vi "Two Way Event Recorder RT Driver VI.vi"(6 "Device Clock":string, 9 "Device Inputs FIFO":refnum<k33>, 10 "Device Outputs FIFO":refnum<k33>, 11 "Device Reference":T1 format="%.0x") -> ()   [LabVIEW 2017, in "Two Way Event Recorder Custom Device.lvlib"]
uses:
  Two Way Event Recorder Custom Device.lvlib
  <vilib>/NI Veristand/Custom Device API/Custom Device Item Ref.ctl
  <vilib>/NI Veristand/Custom Device API/Custom Device Channel Type.ctl
  <vilib>/NI Veristand/Custom Device API/Custom Device Waveform DataType.ctl
  <vilib>/NI Veristand/Custom Device API/Message Response (String).ctl
  <vilib>/NI Veristand/Custom Device API/Message Response (Byte Array).ctl
  <vilib>/NI Veristand/Custom Device Waveform API/Waveform Session.lvclass/Waveform Session.ctl
  <vilib>/NI VeriStand/Custom Device Waveform API/Single Waveform Write (DBL)/Single Waveform Write (DBL).lvclass/Single Waveform Write (DBL).ctl
  <vilib>/NI Veristand/Custom Device Waveform API/Internal Comm Classes/WPL Comm/WPL Comm.lvclass/WPL Comm.ctl
  <vilib>/NI VeriStand/Custom Device Waveform API/Internal Comm Classes/WPL Comm/WPL Comm (1D DBL)/WPL Comm (1D DBL).lvclass/WPL Comm (1D DBL).ctl
  <vilib>/NI Veristand/Custom Device Waveform API/Single Waveform Write (DBL)/NI VeriStand - Start Single Waveform (DBL).vi
  <vilib>/NI Veristand/Custom Device Waveform API/Single Waveform Write (DBL)/NI VeriStand - Write Single Waveform (DBL).vi
  <vilib>/NI Veristand/Custom Device Waveform API/Internal Comm Classes/WPL Comm/WPL_start dbl waveform.vi
  <vilib>/NI Veristand/Custom Device Waveform API/Read Sample offset DVR.vi
  <vilib>/NI Veristand/Custom Device Waveform API/Check Opened.vi
  <vilib>/NI Veristand/Custom Device Waveform API/Internal Comm Classes/WPL Comm/WPL Comm (1D DBL)/Comm_write 1d dbl.vi
  <vilib>/NI Veristand/Custom Device Waveform API/Internal Comm Classes/WPL Comm/Set t0 on Variant.vi
  <vilib>/NI Veristand/Custom Device Waveform API/Internal Comm Classes/WPL Comm/Send WPL Command.vi
  <vilib>/NI Veristand/Custom Device Waveform API/Internal Comm Classes/WPL Comm/Direct Send WPL Command.vi
  <vilib>/NI Veristand/Custom Device Waveform API/Internal Comm Classes/WPL Comm/Convert Q Error to Shutdown Error.vi
  <vilib>/NI VeriStand/Custom Device Waveform API/Single Waveform Write (DBL)/Single Waveform Write (DBL).lvclass
  C:/Program Files (x86)/National Instruments/LabVIEW 2017/vi.lib/NI Veristand/Custom Device Waveform API/Waveform Session.lvclass
  <vilib>/NI VeriStand/Custom Device Waveform API/Internal Comm Classes/WPL Comm/WPL Comm (1D DBL)/WPL Comm (1D DBL).lvclass
  C:/Program Files (x86)/National Instruments/LabVIEW 2017/vi.lib/NI Veristand/Custom Device Waveform API/Internal Comm Classes/WPL Comm/WPL Comm.lvclass
  <vilib>/NI Veristand/Custom Device Waveform API/Single Waveform Write (DBL)/NI VeriStand - Open Single Waveform Write Session (DBL).vi
  <vilib>/Utility/error.llb/Error Cluster From Error Code.vi
  <vilib>/NI Veristand/Custom Device Waveform API/Single Waveform Write (DBL)/NI VeriStand - Close Single Waveform Write Session (DBL).vi
  <vilib>/NI Veristand/Custom Device Tools/Custom Device Utility Library/Custom Device Utility Library.lvlib
  <vilib>/NI Veristand/Custom Device API/Custom Device API.lvlib
  <vilib>/NI Veristand/Custom Device Waveform API/NI_VS Custom Device Waveform API.lvlib
panel:
  in  "Initialization Status Notifier":refnum<notifier>
  in  "Status Notifier":refnum<notifier>
  # "Custom Device Template\nv1.0"
  # "Use this template as a starting point for creating a custom device code module. The input controls shown here are specially named controls that the system will use to provide the device loop with data. The controls are not required for the device loop to run. For instance, if the device doesn't produce any output data, then you don't need the Device Outputs FIFO control. If you do use these controls, however, they need to have these exact names to be functional."
  # "The optional status notifier element is used to notify the RT engine of the last state of the custom device, and to indicate the device has completed execution. If this control is not used, a default No Error value is returned to the system when the device finishes execution.\n\nNote: This error state is not checked until the system shuts down. Use an output status channel to send more immediate status values to the system."
  # "This optional input can be used to send the VeriStand Engine the final status of the custom device initalization process. If this control exists on the custom device front panel, the VeriStand Engine will wait for a status update before starting up. If the custom device reports an error, that will abort the execution of the current configuration in the VeriStand Engine.\n\nThis control can be deleted if the custom device does not need to send the initialization status update."
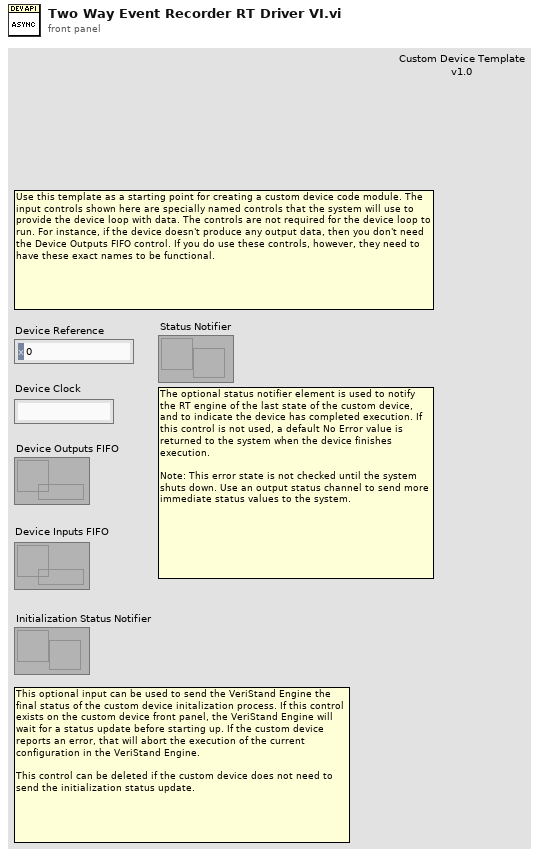
[diagram p1: front panel]
types:
  T1 = typedef "Custom Device API.lvlib/Custom Device Item Ref.ctl" = u64
  T2 = typedef "Custom Device API.lvlib/Custom Device Channel Type.ctl" = enum16{"Input", "Output"}
  T3 = typedef "Custom Device API.lvlib/Custom Device Waveform DataType.ctl" = enum16{"Double", "Complex Double"}
  T4 = typedef "Custom Device API.lvlib/Custom Device Engine Event Ref.ctl" = refnum<event-registration>
  T5 = typedef "Custom Device API.lvlib/Waveform Data Reference.ctl" = i32
  T6 = typedef "Custom Device API.lvlib/Message Response (String).ctl" = cluster{"Response":string, "Error":errorcluster}
  T7 = typedef "Custom Device API.lvlib/Message Response (Byte Array).ctl" = cluster{"Response":u8[], "Error":errorcluster}
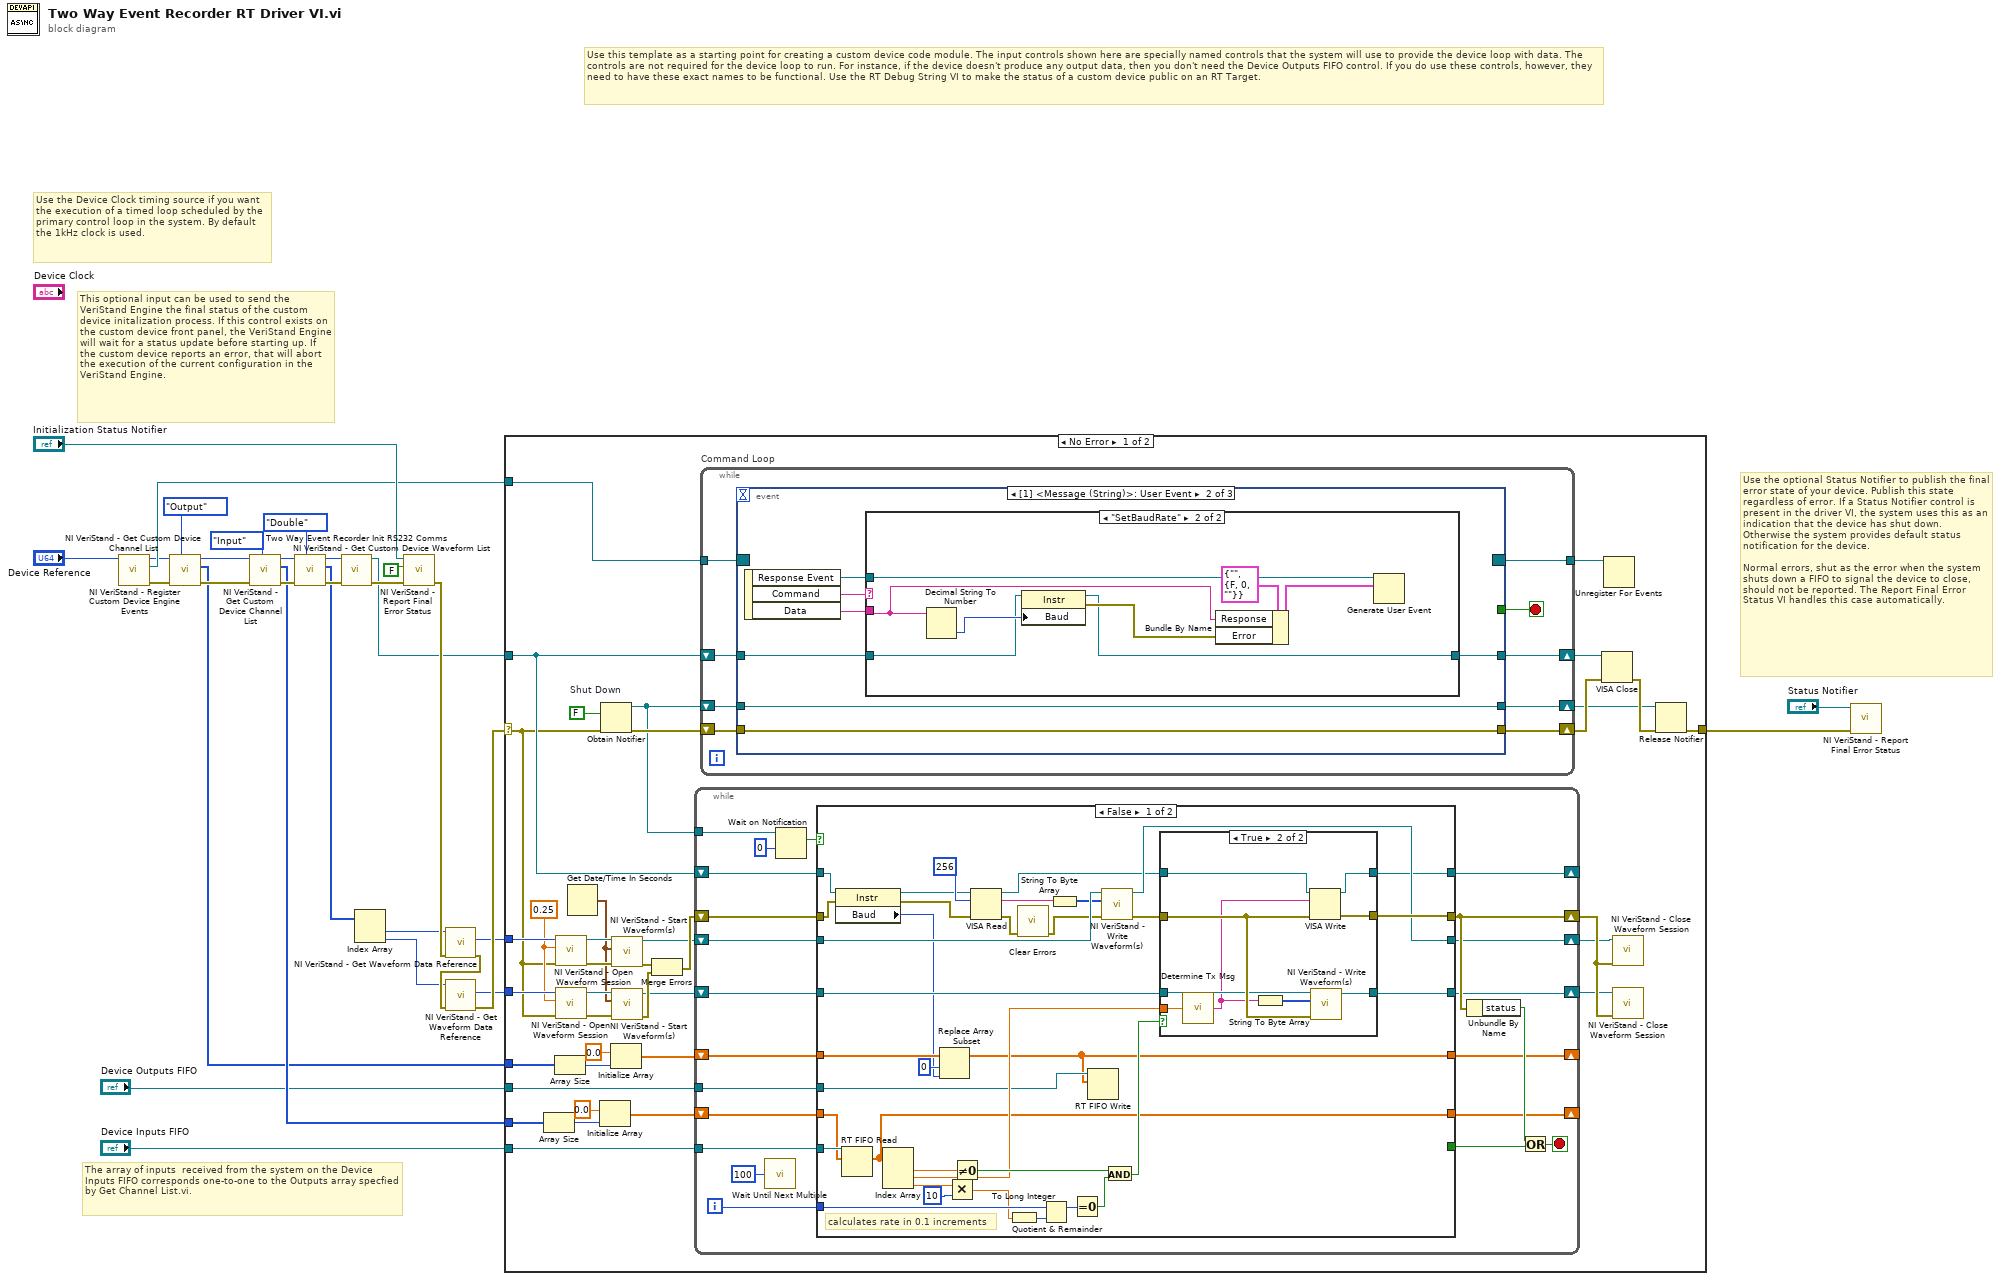
[diagram p0: block diagram]
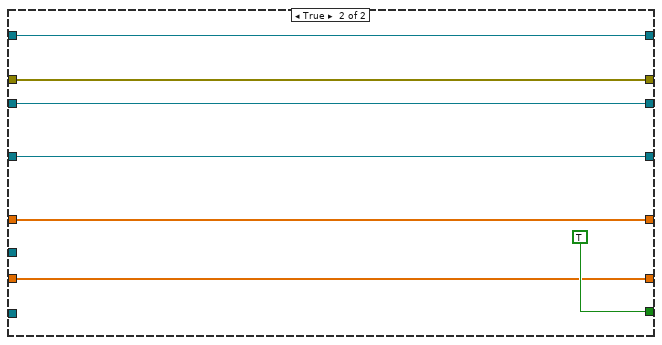
[diagram p3: hidden frame]
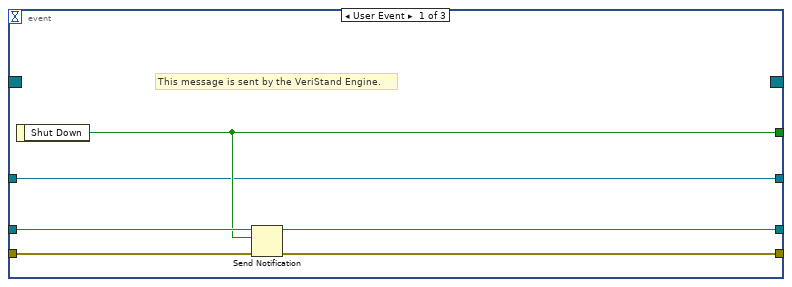
[diagram p4: hidden frame]
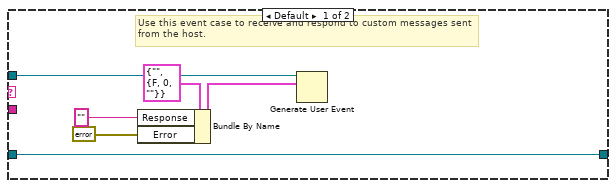
[diagram p5: hidden frame]
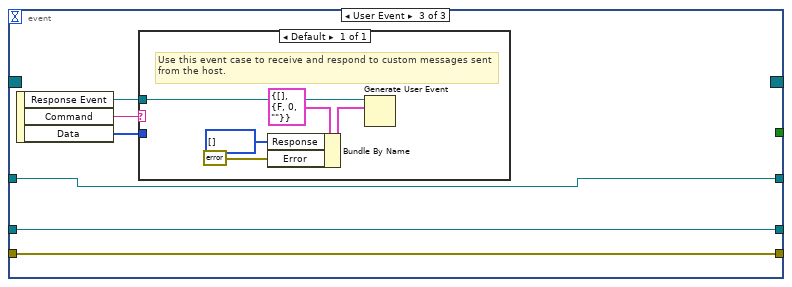
[diagram p6: hidden frame]
diagram:
  # "This optional input can be used to send the VeriStand Engine the final status of the custom device initalization process. If this control exists on the custom device front panel, the VeriStand Engine will wait for a status update before starting up. If the custom device reports an error, that will abort the execution of the current configuration in the VeriStand Engine."
  # "The array of inputs  received from the system on the Device Inputs FIFO corresponds one-to-one to the Outputs array specfied by Get Channel List.vi."
  # "Use the optional Status Notifier to publish the final error state of your device. Publish this state regardless of error. If a Status Notifier control is present in the driver VI, the system uses this as an indication that the device has shut down. Otherwise the system provides default status notification for the device.\n\nNormal errors, shut as the error when the system shuts down a FIFO to signal the device to close, should not be reported. The Report Final Error Status VI handles this case automatically."
  # "Use the Device Clock timing source if you want the execution of a timed loop scheduled by the primary control loop in the system. By default the 1kHz clock is used."
  # "Use this template as a starting point for creating a custom device code module. The input controls shown here are specially named controls that the system will use to provide the device loop with data. The controls are not required for the device loop to run. For instance, if the device doesn't produce any output data, then you don't need the Device Outputs FIFO control. If you do use these controls, however, they need to have these exact names to be functional. Use the RT Debug String VI to make the status of a custom device public on an RT Target."
  n1 = call <vilib>:"NI VeriStand - Register Custom Device Engine Events.vi"("Device Ref in"="Device Reference") -> ("error out"=w6:errorcluster, "Custom Device Engine Event Ref"=w21:T4, "Device Ref out"=w7:T1)  [unwired: 8 in]
  n2 = call <vilib>:"NI VeriStand - Get Custom Device Channel List.vi"("Channel Type"=Custom_Device_Channel_Type."Output", "error in (no error)"=w6, "Device Ref in"=w7) -> ("error out"=w5:errorcluster, "Specified Channel Ref List"=w1:T1[], "Device Ref out"=w4:T1)  [unwired: 6 in]
  n3 = call <vilib>:"NI VeriStand - Get Custom Device Channel List.vi"("Channel Type"=Custom_Device_Channel_Type."Input", "error in (no error)"=w5, "Device Ref in"=w4) -> ("error out"=w27:errorcluster, "Specified Channel Ref List"=w17:T1[], "Device Ref out"=w14:T1)  [unwired: 6 in]
  n4 = call <vilib>:"NI VeriStand - Get Custom Device Waveform List.vi"("Waveform Data Type"=Custom_Device_Waveform_DataType."Double", "error in (no error)"=w27, "Device Ref in"=w14) -> ("error out"=w26:errorcluster, "Specified Waveform Ref List"=w15:T1[], "Device Ref out"=w13:T1)  [unwired: 6 in]
  n5 = call "Two Way Event Recorder Init RS232 Comms.vi"("error in (no error)"=w26, "Device Ref in"=w13) -> ("error out"=w28:errorcluster, "Visa reference out"=w20:refnum<visa-resource-name>)  [unwired: 8 in]
  n6 = Index Array(array=w15) -> (element #1=w12:T1, element #2=w10:T1)  [unwired: 2 in]
  n7 = call <vilib>:"NI VeriStand - Report Final Error Status.vi"("error in (no error)"=w28, "Filter FIFO & Shutdown Errors (T)"=FALSE ("Filter FIFO Errors (T)"), "Status Notifier"="Initialization Status Notifier") -> ("error out"=w29:errorcluster)  [unwired: 8 out]
  n8 = call <vilib>:"NI VeriStand - Get Waveform Data Reference.vi"("error in (no error)"=w29, "Waveform Ref in"=w12) -> ("error out"=w30:errorcluster, "Waveform Data Reference"=w11:T5)  [unwired: 7 in, 1 out]
  n9 = call <vilib>:"NI VeriStand - Get Waveform Data Reference.vi"("error in (no error)"=w30, "Waveform Ref in"=w10) -> ("error out"=w31:errorcluster, "Waveform Data Reference"=w8:T5)  [unwired: 7 in, 1 out]
  n10 = case shown="No Error" w31 {
    selector: w31 -> [w41 w194]
    tunnel: w21 -> [w64 _]
    tunnel: [w62 w194] -> w9
    tunnel: w20 -> [w42 _]
    tunnel: "Device Inputs FIFO" -> [w57 _]
    tunnel: w17 -> [w37 _]
    tunnel: w11 -> [w55 _]
    tunnel: w8 -> [w49 _]
    tunnel: "Device Outputs FIFO" -> [w40 _]
    tunnel: w1 -> [w33 _]
    frame No Error {
      w44 = 0.25 ("dt")
      w63 = FALSE  # Shut Down
      n11 = Array Size(array=w37) -> (size(s)=w39:i32)
      n12 = Array Size(array=w33) -> (size(s)=w35:i32)
      n13 = call-poly <vilib>:"NI VeriStand - Open Waveform Session.vi"("error in (no error)"=w41, "dt"=w44, "DBL Waveform Data Reference"=w55) -> ("error out"=w56:errorcluster, "Single Waveform Write Session (DBL)"=w54:refnum<class "Single Waveform Write (DBL).lvclass">)  [unwired: 7 in]
      n14 = call-poly <vilib>:"NI VeriStand - Open Waveform Session.vi"("error in (no error)"=w41, "dt"=w44, "DBL Waveform Data Reference"=w49) -> ("error out"=w50:errorcluster, "Single Waveform Write Session (DBL)"=w51:refnum<class "Single Waveform Write (DBL).lvclass">)  [unwired: 7 in]
      n15 = Get Date/Time In Seconds() -> (seconds since 1Jan1904=w46:timestamp)
      n16 = Initialize Array(0.0 ("element"), w39) -> (w36:dbl[])
      n17 = Obtain Notifier(notification data type=w63, error in (no error)=w41) -> (notifier out=w58:refnum<notifier>, error out=w65:errorcluster)  [unwired: 2 in, 1 out]
      n18 = Initialize Array(0.0 ("element"), w35) -> (w32:dbl[])
      n19 = call-poly <vilib>:"NI VeriStand - Start Waveform(s).vi"("error in (no error)"=w56, "t0"=w46, "Single Waveform Write Session (DBL) in"=w54) -> ("error out"=w48:errorcluster, "Single Waveform Write Session (DBL) out"=w53:refnum<class "Single Waveform Write (DBL).lvclass">)  [unwired: 7 in]
      n20 = call-poly <vilib>:"NI VeriStand - Start Waveform(s).vi"("error in (no error)"=w50, "t0"=w46, "Single Waveform Write Session (DBL) in"=w51) -> ("error out"=w47:errorcluster, "Single Waveform Write Session (DBL) out"=w45:refnum<class "Single Waveform Write (DBL).lvclass">)  [unwired: 7 in]
      n21 = Merge Errors(w48, w47) -> (w68:errorcluster)
      n22 = while {
        shift-right: [w88] -> w69
        shift-left: w68 -> [w90]
        shift-right: [w89] -> _
        shift-left: w42 -> [w91]
        tunnel: w58 -> [w84]
        tunnel: w57 -> [w80]
        shift-right: [w78] -> w52
        shift-left: w53 -> [w79]
        shift-right: [w76] -> w43
        shift-left: w45 -> [w77]
        tunnel: w40 -> [w74]
        shift-right: [w72] -> _
        shift-left: w36 -> [w73]
        shift-right: [w70] -> _
        shift-left: w32 -> [w71]
        i -> [w75]
        stop <- w86 stop-if-true
        n23 = call "Wait Until Next Multiple"("Count(mSec)"=u32 100) -> ()  [unwired: 1 out]
        n24 = Wait on Notification(notifier=w84, timeout in ms (-1)=0) -> (notification=w83:bool)  [unwired: 2 in, 3 out]
        n25 = case shown="False" w83 {
          tunnel: w91 -> [w97 w145]
          tunnel: w90 -> [w95 w144]
          tunnel: [w127 w144] -> w88
          tunnel: [w125 w145] -> w89
          tunnel: [_ TRUE ("y")] -> w85
          tunnel: w80 -> [w124 _]
          tunnel: w73 -> [w123 w140]
          tunnel: w79 -> [w119 w143]
          tunnel: [w126 w143] -> w78
          tunnel: w77 -> [w113 w142]
          tunnel: [w112 w142] -> w76
          tunnel: w75 -> [w107 _]
          tunnel: w74 -> [w101 _]
          tunnel: w71 -> [w100 w141]
          tunnel: [w99 w140] -> w72
          tunnel: [w92 w141] -> w70
          frame False {
            # "calculates rate in 0.1 increments"
            n26 = property class="Instr"(reference=w97, error in=w95) -> (reference out=w96:refnum<visa-resource-name>, error out=w94:errorcluster, "Baud"=w93:u32)
            n27 = RT FIFO Read(0:w124, 1:w123) -> (9:w99:dbl[])  [unwired: 2 in, 4 out]
            n28 = Index Array(array=w99) -> (element #1=w122:dbl, element #2=w114:dbl, element #3=w105:dbl)  [unwired: 3 in]
            n29 = Replace Array Subset(array=w100, new element=w93, index=0) -> (w92:dbl[])
            n30 = Multiply(x=w105, y=10) -> (x*y=w103:dbl)
            n31 = Not Equal To 0?(x=w122) -> (x != 0?=w115:bool)
            n32 = VISA Read(VISA resource name=w96, byte count=u32 256, error in (no error)=w94) -> (VISA resource name out=w117:refnum<visa-resource-name>, read buffer=w118:string, error out=w110:errorcluster)  [unwired: 1 out]
            n33 = To Long Integer(number=w103) -> (32bit integer=w102:i32)
            n34 = call <vilib>:"Clear Errors.vi"("error in (no error)"=w110) -> ("error out"=w109:errorcluster)  [unwired: 5 in, 1 out]
            n35 = Quotient & Remainder(x=w107, y=w102) -> (x-y*floor(x/y)=w108:i32)  [unwired: 1 out]
            n36 = String To Byte Array(string=w118) -> (unsigned byte array=w111:u8[])
            n37 = Equal To 0?(x=w108) -> (x = 0?=w106:bool)
            n38 = RT FIFO Write(0:w101, 1:w92) -> ()  [unwired: 3 in, 4 out]
            n39 = call-poly <vilib>:"NI VeriStand - Write Waveform(s).vi"("error in (no error)"=w109, "Data"=w111, "Single Waveform Write Session (DBL) in"=w119) -> ("error out"=w121:errorcluster, "Single Waveform Write Session (DBL) out"=w126:refnum<class "Single Waveform Write (DBL).lvclass">)  [unwired: 6 in, 1 out]
            n40 = And(x=w115, y=w106) -> (x .and. y?=w116:bool)
            n41 = case shown="True" w116 {
              tunnel: w117 -> [w130 w138]
              tunnel: w121 -> [w129 w139]
              tunnel: [w130 w137] -> w125
              tunnel: [w129 w135] -> w127
              tunnel: w114 -> [_ w136]
              tunnel: w113 -> [w128 w134]
              tunnel: [w128 w133] -> w112
              frame False {
              }
              frame True {
                n42 = call "Determine Tx Msg.vi"("Tx Msg Type"=w136) -> ("Tx String"=w131:string)
                n43 = String To Byte Array(string=w131) -> (unsigned byte array=w132:u8[])
                n44 = VISA Write(VISA resource name=w138, write buffer=w131, error in (no error)=w139) -> (VISA resource name out=w137:refnum<visa-resource-name>, error out=w135:errorcluster)  [unwired: 1 out]
                n45 = call-poly <vilib>:"NI VeriStand - Write Waveform(s).vi"("error in (no error)"=w139, "Data"=w132, "Single Waveform Write Session (DBL) in"=w134) -> ("Single Waveform Write Session (DBL) out"=w133:refnum<class "Single Waveform Write (DBL).lvclass">)  [unwired: 6 in, 2 out]
              }
            }
          }
          frame True {
          }
        }
        n46 = Unbundle By Name(w88) -> ("status"=w87:bool)
        n47 = Or(x=w87, y=w85) -> (x .or. y?=w86:bool)
      }
      n48 = while "Command Loop" {
        tunnel: w64 -> [w155]
        tunnel: [w154] -> w61
        shift-right: [w151] -> w60
        shift-left: w58 -> [w152]
        shift-right: [w149] -> w67
        shift-left: w65 -> [w150]
        shift-right: [w147] -> w59
        shift-left: w42 -> [w148]
        stop <- w153 stop-if-true
        n49 = event shown="[1] <Message (String)>: User Event" {
          selector: w155 -> [_ _ _]
          dyn-events: [_ _ _] -> w154
          timeout: _ -> [_ _ _]
          tunnel: [w159 _ _] -> w153
          tunnel: w152 -> [w160 w166 w186]
          tunnel: [w161 w166 w186] -> w151
          tunnel: w150 -> [w158 w163 w184]
          tunnel: [w157 w163 w184] -> w149
          tunnel: w148 -> [w156 w164 w183]
          tunnel: [w156 w162 w183] -> w147
          event User Event {
            # "This message is sent by the VeriStand Engine."
            n50 = event-data() -> ("Shut Down"=w159:bool)  [unwired: 1 in]
            n51 = Send Notification(notification=w159, notifier=w160, error in (no error)=w158) -> (notifier out=w161:refnum<notifier>, error out=w157:errorcluster)
          }
          event User Event {
            n52 = event-data() -> ("Response Event"=w165:refnum<user-event>, "Command"=w168:string, "Data"=w167:string)  [unwired: 1 in]
            n53 = case shown="\"SetBaudRate\"" w168 {
              tunnel: w167 -> [_ w175]
              tunnel: w165 -> [w174 w182]
              tunnel: w164 -> [w169 w178]
              tunnel: [w169 w176] -> w162
              frame Default {
                # "Use this event case to receive and respond to custom messages sent from the host."
                n54 = Bundle By Name(cluster=T6 {"Response"="", "Error"={"status"=FALSE, "code"=0, "source"=""}} ("event data"), "Response"="", "Error"=errorcluster {"status"=FALSE, "code"=0, "source"=""}) -> (w172:T6)
                n55 = Generate User Event(user event=w174, event data cluster=w172) -> ()  [unwired: 2 in, 2 out]
              }
              frame "SetBaudRate" {
                n56 = Decimal String To Number(string=w175) -> (number=w179:i32)  [unwired: 2 in, 1 out]
                n57 = property class="Instr"(reference=w178, "Baud"=w179) -> (reference out=w176:refnum<visa-resource-name>, error out=w177:errorcluster)  [unwired: 1 in]
                n58 = Bundle By Name(cluster=T6 {"Response"="", "Error"={"status"=FALSE, "code"=0, "source"=""}} ("event data"), "Response"=w175, "Error"=w177) -> (w180:T6)
                n59 = Generate User Event(user event=w182, event data cluster=w180) -> ()  [unwired: 2 in, 2 out]
              }
            }
          }
          event User Event {
            n60 = event-data() -> ("Response Event"=w185:refnum<user-event>, "Command"=w188:string, "Data"=w187:u8[])  [unwired: 1 in]
            n61 = case shown="Default" w188 {
              tunnel: w187 -> [_]
              tunnel: w185 -> [w193]
              frame Default {
                # "Use this event case to receive and respond to custom messages sent from the host."
                n62 = Bundle By Name(cluster=T7 {"Response"=[], "Error"={"status"=FALSE, "code"=0, "source"=""}} ("event data"), "Response"=u8[] [], "Error"=errorcluster {"status"=FALSE, "code"=0, "source"=""}) -> (w190:T7)
                n63 = Generate User Event(user event=w193, event data cluster=w190) -> ()  [unwired: 2 in, 2 out]
              }
            }
          }
        }
      }
      n64 = VISA Close(VISA resource name=w59, error in (no error)=w67) -> (error out=w66:errorcluster)
      n65 = Unregister For Events(event registration refnum=w61) -> ()  [unwired: 1 in, 1 out]
      n66 = call-poly <vilib>:"NI VeriStand - Close Waveform Session.vi"("error in (no error)"=w69, "Single Waveform Write Session (DBL)"=w52) -> ()  [unwired: 9 in, 1 out]
      n67 = call-poly <vilib>:"NI VeriStand - Close Waveform Session.vi"("error in (no error)"=w69, "Single Waveform Write Session (DBL)"=w43) -> ()  [unwired: 9 in, 1 out]
      n68 = Release Notifier(notifier=w60, error in (no error)=w66) -> (error out=w62:errorcluster)  [unwired: 1 in, 2 out]
    }
    frame Error {
    }
  }
  n69 = call <vilib>:"NI VeriStand - Report Final Error Status.vi"("error in (no error)"=w9, "Status Notifier"="Status Notifier") -> ()  [unwired: 1 in, 9 out]
